vi "Play Path.vi"(7 "Description":string, 8 "Command Info In":T6, 11 "Auto Data":T5) -> (0 "Command Info Out":T6)   [LabVIEW 2023]
doc: "This VI notifies the subsystem to the new setpoint."
uses:
  <vilib>/Rock Robotics/WPI/Framework/Command Status Info.ctl
  <vilib>/Rock Robotics/WPI/Framework/Completion Status.ctl
  <vilib>/Rock Robotics/WPI/Framework/Completion Notifier.ctl
  bordeaux-main/Bordeaux/Types/Single Cmd Info.ctl
  <vilib>/picture/picture.llb/imagedata.ctl
  bordeaux-main/Bordeaux/Types/Trajectory Data.ctl
  bordeaux-main/Bordeaux/Types/Segment Type.ctl
  Implementation/Drive Setpoints.ctl
  Implementation/Drive Operations.ctl
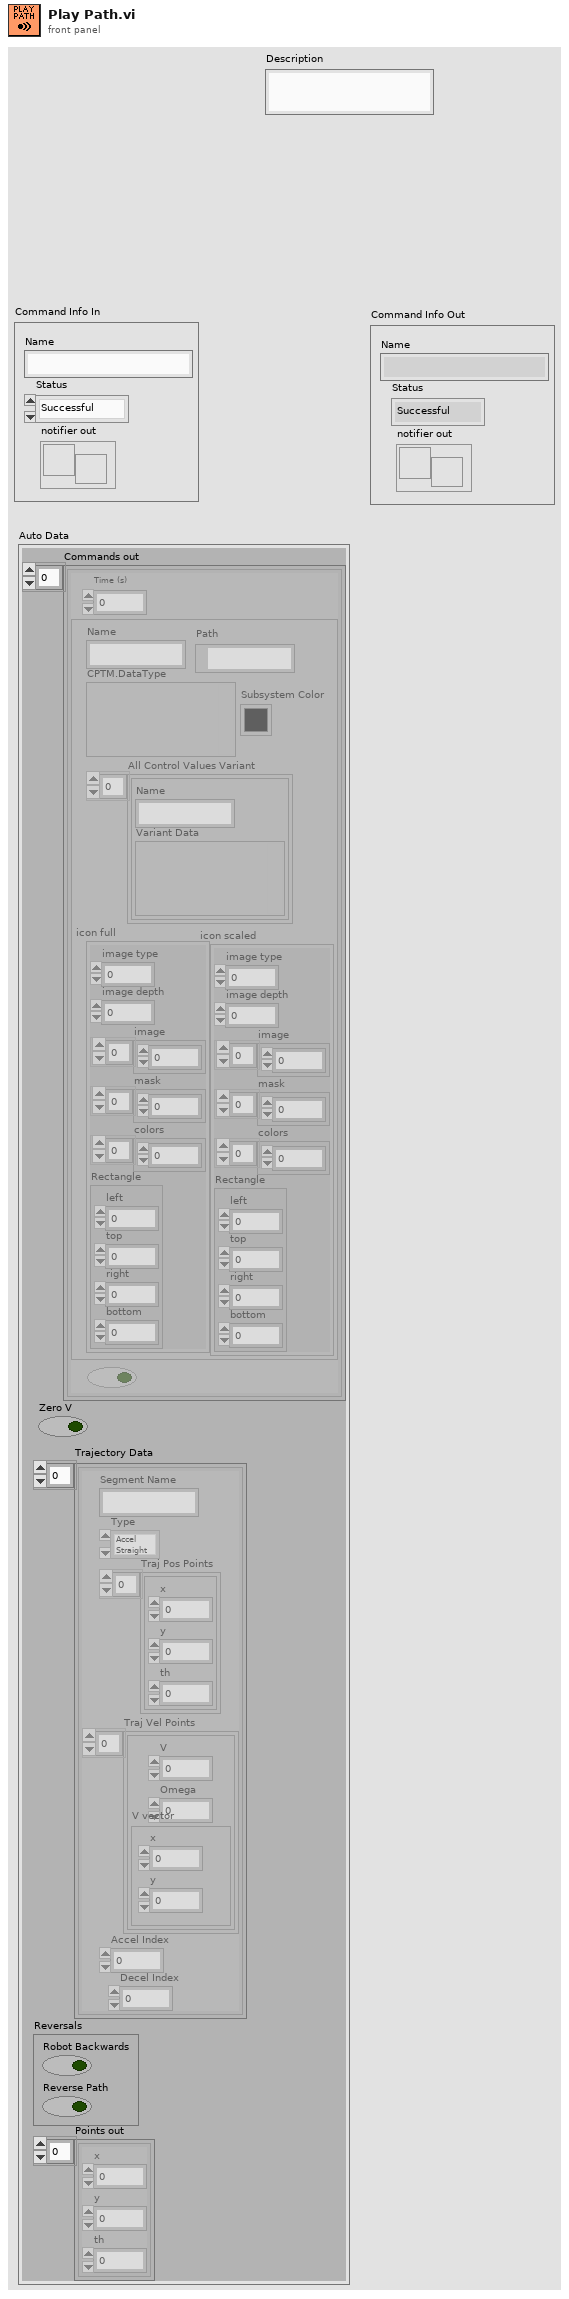
[diagram p1: front panel]
types:
  T1 = typedef "Single Cmd Info.ctl" = cluster{"Name":string, "CPTM.DataType":variant, "All Control Values Variant":cluster{"Name":string, "Variant Data":variant}[], "icon full":T2, "icon scaled":T2, "Path":path, "Subsystem Color":u32}
  T2 = typedef "imagedata.ctl" = cluster{"image type":i32, "image depth":i32, "image":u8[], "mask":u8[], "colors":u32[], "Rectangle":cluster{"left":i16, "top":i16, "right":i16, "bottom":i16}}
  T3 = typedef "Trajectory Data.ctl" = cluster{"Segment Name":string, "Type":T4, "Traj Pos Points":cluster{"x":dbl, "y":dbl, "th":dbl}[], "Traj Vel Points":cluster{"V":dbl, "Omega":dbl, "V vector":cluster{"y":dbl, "x":dbl}}[], "Accel Index":i32, "Decel Index":i32}[]
  T4 = typedef "Segment Type.ctl" = enum16{"Accel Straight", "Const Straight", "Blend", "Circle", "Bezier"}
  T5 = cluster{"Commands out":cluster{"Time (s)":dbl, T1, bool}[], "Zero V":bool, "Trajectory Data":T3, "Reversals":cluster{"Robot Backwards":bool, "Reverse Path":bool}, "Points out":cluster{"x":dbl, "y":dbl, "th":dbl}[]}
  T6 = typedef "Command Status Info.ctl" = cluster{"Name":string, "Status":T7, "notifier out":T8}
  T7 = typedef "Completion Status.ctl" = enum16{"Successful", "Aborted", "Incomplete"}
  T8 = typedef "Completion Notifier.ctl" = refnum<notifier>
  T9 = typedef "Drive Setpoints.ctl" = cluster{"Operation":T10, "Left Setpoint":dbl, "Right Setpoint":dbl, "Duration":dbl, "Auto Data":cluster{"Commands out":cluster{"Time (s)":dbl, T1, bool}[], "Zero V":bool, "Trajectory Data":T3, "Reversals":cluster{"Robot Backwards":bool, "Reverse Path":bool}, "Points out":cluster{"x":dbl, "y":dbl, "th":dbl}[]}}
  T10 = typedef "Drive Operations.ctl" = enum16{"Reserve", "Read Current", "Immediate", "Drive for Time", "Play Path", "Drive for Distance"}
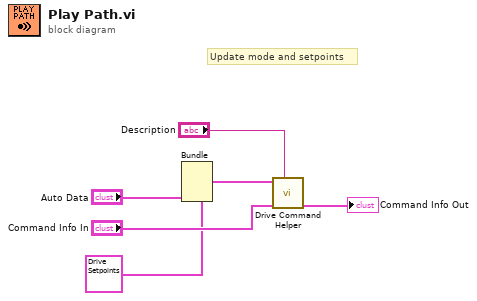
[diagram p0: block diagram]
diagram:
  # "Update mode and setpoints"
  n1 = Bundle(cluster=T9 {"Operation"=enum."Play Path", "Left Setpoint"=0.0, "Right Setpoint"=0.0, "Duration"=0.0, "Auto Data"={"Commands out"=[], "Zero V"=FALSE, "Trajectory Data"=[], "Reversals"={"Robot Backwards"=FALSE, "Reverse Path"=FALSE}, "Points out"=[]}} ("SubSystem Data"), "Auto Data"="Auto Data") -> (w2:T9)  [unwired: 4 in]
  n2 = call "Drive Command Helper.vi"("Description"="Description", "Command Info In"="Command Info In", "SubSystem Data"=w2) -> ("Command Info Out"=→"Command Info Out":T6)  [unwired: 6 in, 2 out]
